vi "Collect.vi"(8 "error in (no error)":errorcluster, 11 "Disk Collector in":refnum<class "Disk Collector.lvclass">) -> (0 "error out":errorcluster, 2 "Metrics":refnum<data-value>[](array[refnum]), 3 "Disk Collector out":refnum<class "Disk Collector.lvclass">)   [LabVIEW 2020, in "Disk Collector.lvclass"]
uses:
  Disk Collector.lvclass
  C:/Github-locals/PromVIEW/src/collector/generic collector/Default Collector.lvclass
  src/metrics/metric/Metric.lvclass
  src/metrics/gauge/Gauge.lvclass
  Disk Collector.lvclass/Disk Collector.ctl
  src/collector/generic collector/Default Collector.lvclass
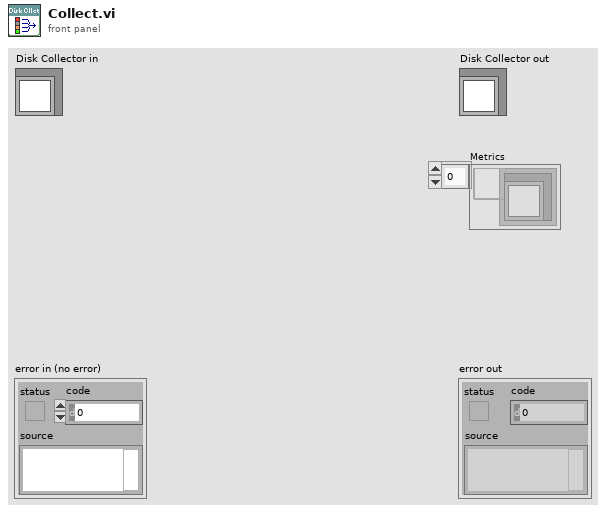
[diagram p1: front panel]
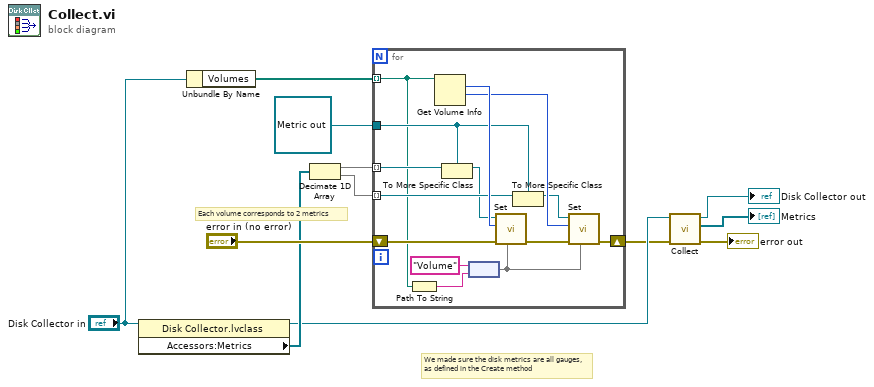
[diagram p0: block diagram]
diagram:
  # "We made sure the disk metrics are all gauges, as defined in the Create method"
  # "Each volume corresponds to 2 metrics"
  n1 = property class="Disk Collector.lvclass"(reference="Disk Collector in") -> (reference out=w3:refnum<class "Disk Collector.lvclass">, "Accessors:Metrics"=w5:refnum<data-value>[])  [unwired: 1 in, 1 out]
  n2 = Unbundle By Name("Disk Collector in") -> ("Volumes"=w10:path[])
  n3 = Decimate 1D Array(w5) -> (w9:refnum<data-value>[], w8:refnum<data-value>[])
  n4 = for {
    tunnel: w10 -> [w14] mode=indexing
    tunnel: w9 -> [w21] mode=indexing
    tunnel: w8 -> [w20] mode=indexing
    shift-right: [w22] -> w1
    shift-left: "error in (no error)" -> [w23]
    tunnel: refnum<data-value> refnum ("Gauge Ref") -> [w19]
    n5 = Path To String(path=w14) -> (string=w15:string)
    n6 = Get Volume Info(11:w14) -> (1:w25:i64, 2:w26:i64)  [unwired: 1 in, 4 out]
    n7 = To More Specific Class(target class=w19, reference=w21) -> (specific class reference=w18:refnum<data-value>)  [unwired: 1 in, 1 out]
    n8 = node("Volume" ("key"), w15) -> (w13:map{string, string})
    n9 = call "Set.vi"("Labels"=w13, "error in (no error)"=w23, "Value"=w26, "Gauge Ref"=w18) -> ("error out"=w24:errorcluster)  [unwired: 6 in, 1 out]
    n10 = To More Specific Class(target class=w19, reference=w20) -> (specific class reference=w17:refnum<data-value>)  [unwired: 1 in, 1 out]
    n11 = call "Set.vi"("Labels"=w13, "error in (no error)"=w24, "Value"=w25, "Gauge Ref"=w17) -> ("error out"=w22:errorcluster)  [unwired: 6 in, 1 out]
  }
  n12 = call-parent "Collect.vi"("error in (no error)"=w1, "Default Collector in"=w3) -> ("error out"=→"error out":errorcluster, "Metrics"=→"Metrics":refnum<data-value>[], "Default Collector out"=→"Disk Collector out":refnum<class "Disk Collector.lvclass">)  [unwired: 7 in]
